vi "Main Page.vi"(8 "error in (no error)":errorcluster, 11 "Node Ptr":T1 format="%.0x") -> (0 "error out":errorcluster)   [LabVIEW 2020, in "FPGA Addon System Explorer.lvlib"]
uses:
  FPGA Addon System Explorer.lvlib
  <vilib>/NI VeriStand/Custom Device API/Custom Device API.lvlib
  Addon Shared/FPGA Addon Shared.lvlib
  Addon Shared/Types/FG Action.ctl
  <vilib>/NI/NI VeriStand Hardware Resource Discovery/NIVS Hardware Discovery.lvlib
  <vilib>/NI/NI VeriStand Hardware Resource Discovery/_Types/Filter Type.ctl
  <vilib>/NI VeriStand/Custom Device API/Custom Device Item Ref.ctl
panel:
  in  "Refresh bitfile":bool
  out "Group?":bool
  in  "RIO Browse":bool
  out "Version":string
  in  "SHDocVw.IWebBrowser":refnum<k7>(container)
  in  "RIO Device":string
  in  "Bitfile path":path
  in  "Header 2":cluster{"Section Name":string}={"Section Name"="FPGA Settings"}
  in  "Header":cluster{"Section Name":string}={"Section Name"="Addon Settings"}
  in  "Description":string
  in  "Name":string
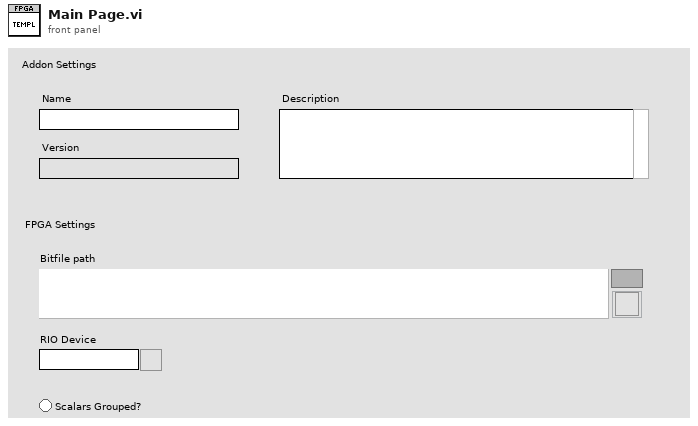
[diagram p1: front panel]
types:
  T1 = typedef "Custom Device API.lvlib/Custom Device Item Ref.ctl" = u64
  T2 = typedef "FPGA Addon Shared.lvlib/FG Action.ctl" = enum8{"GET", "SET"}
  T3 = typedef "FPGA Addon Shared.lvlib/FPGA Settings.ctl" = cluster{"Bitfile path":path, "RIO Device Address":string, "Group":bool}
  T4 = typedef "Custom Device API.lvlib/Custom Device Item Info.ctl" = cluster{"Name":string, "Is Channel":bool, "GUID":string, "Is Waveform":bool}
  T5 = typedef "NIVS Hardware Discovery.lvlib/Filter Type.ctl" = enum16{"Device Category", "Product Name", "Ethernet", "XNET", "VISA", "FPGA", "EtherCAT Master", "DAQmx", "GPIB", "Serial"}
  T6 = typedef "Custom Device API.lvlib/Custom Device Commands.ctl" = enum16{"Default", "Item renamed", "Shutdown", "Dynamic button pressed"}
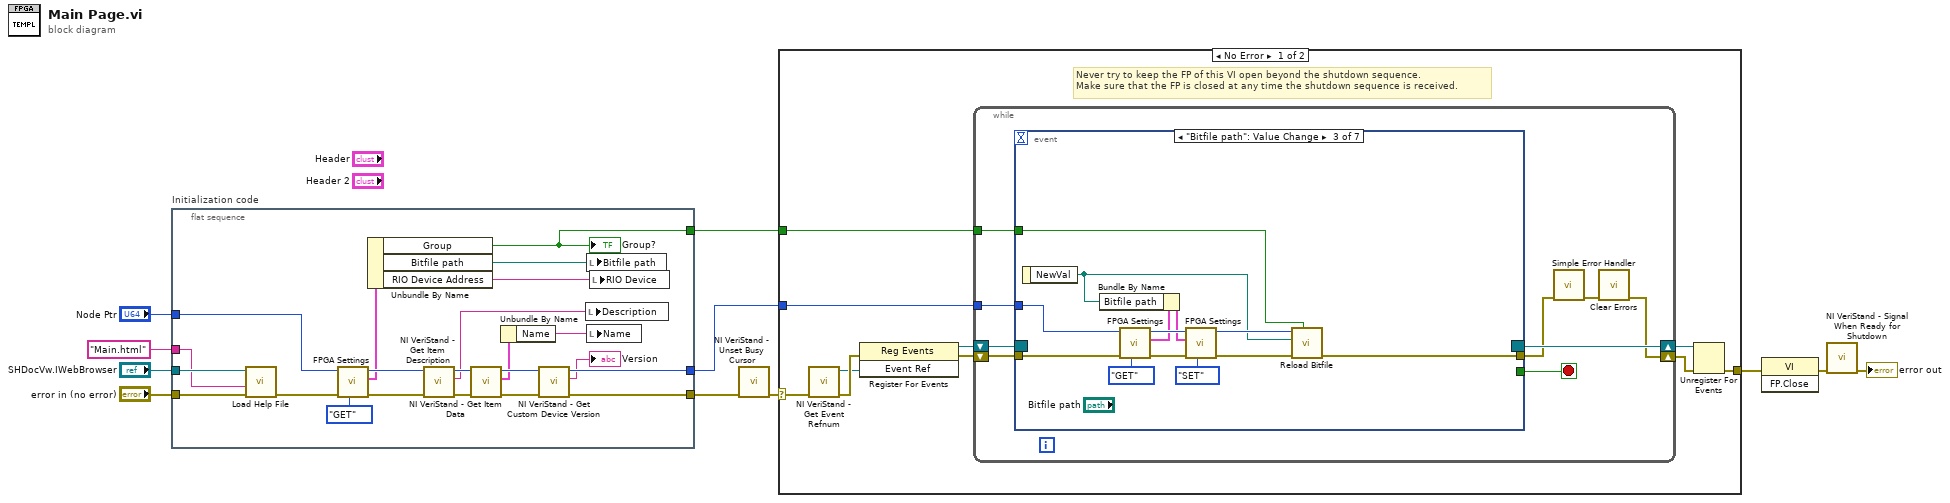
[diagram p0: block diagram]
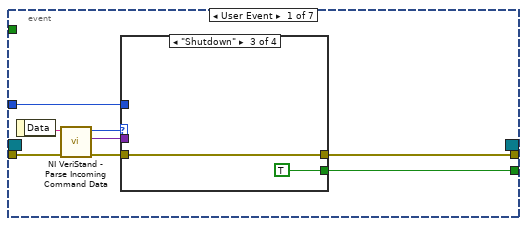
[diagram p2: hidden frame]
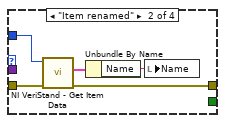
[diagram p4: hidden frame]
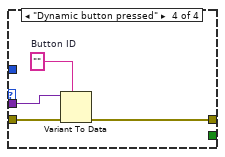
[diagram p5: hidden frame]
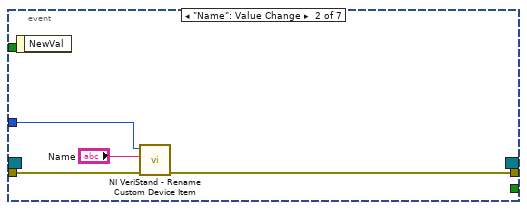
[diagram p6: hidden frame]
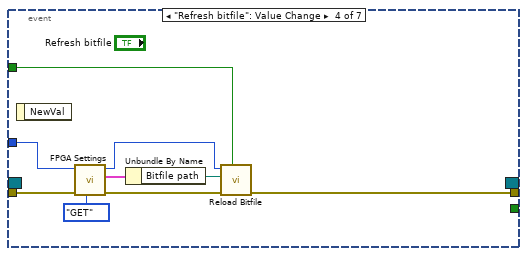
[diagram p7: hidden frame]
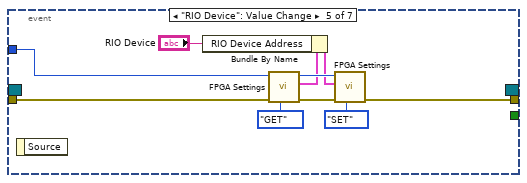
[diagram p8: hidden frame]
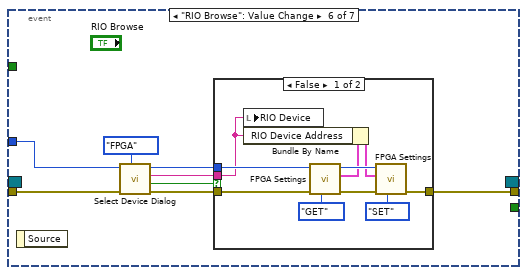
[diagram p9: hidden frame]
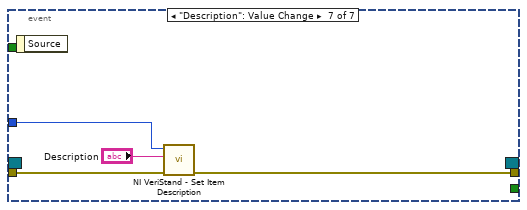
[diagram p11: hidden frame]
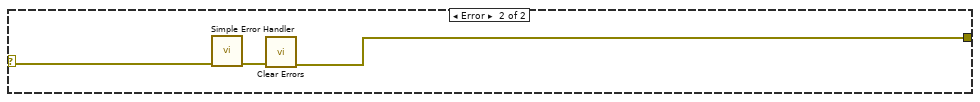
[diagram p12: hidden frame]
diagram:
  n1 = flat-sequence "Initialization code" {
    tunnel: "error in (no error)" -> [w27]
    tunnel: "Node Ptr" -> [w24]
    tunnel: [w15] -> w7
    tunnel: [w16] -> w4
    tunnel: "SHDocVw.IWebBrowser" -> [w26]
    tunnel: "Main.html" ("HTML File") -> [w25]
    tunnel: [w12] -> w1
    frame #0 {
      n2 = call "Load Help File.vi"("error in (no error)"=w27, "HTML File to Load"=w25, "SHDocVw.IWebBrowser2"=w26) -> ("error out"=w23:errorcluster)  [unwired: 8 in]
      n3 = call "FPGA Settings.vi"("Action"=FG_Action."GET", "error in (no error)"=w23, "Item Ref"=w24) -> ("error out"=w21:errorcluster, "FPGA Settings"=w19:T3, "Item Ref out"=w22:T1)  [unwired: 6 in]
      n4 = Unbundle By Name(w19) -> ("Group"=w12:bool, "Bitfile path"=w17:path, "RIO Device Address"=w18:string)
      "Group?" <- w12
      n5 = call <vilib>:"NI VeriStand - Get Item Description.vi"("error in (no error)"=w21, "Item Ref in"=w22) -> ("error out"=w30:errorcluster, "Description"=w31:string, "Item Ref out"=w32:T1)  [unwired: 7 out]
      n6 = call <vilib>:"NI VeriStand - Get Item Data.vi"("error in (no error)"=w30, "Item Ref in"=w32) -> ("error out"=w14:errorcluster, "Item Info"=w29:T4, "Item Ref out"=w33:T1)  [unwired: 7 out]
      n7 = Unbundle By Name(w29) -> ("Name"=w28:string)
      n8 = call <vilib>:"NI VeriStand - Get Custom Device Version.vi"("error in (no error)"=w14, "Device Ref in"=w33) -> ("error out"=w15:errorcluster, "Value"=→"Version":string, "Device Ref out"=w16:T1)  [unwired: 7 in]
      n9 = local write "Description"(w31) -> ()
      n10 = local write "Bitfile path"(w17) -> ()
      n11 = local write "Name"(w28) -> ()
      n12 = local write "RIO Device"(w18) -> ()
    }
  }
  n13 = call <vilib>:"NI VeriStand - Unset Busy Cursor.vi"("error in (no error)"=w7) -> ("error out"=w6:errorcluster)  [unwired: 10 out]
  n14 = case shown="No Error" w6 {
    selector: w6 -> [w35 w134]
    tunnel: [w40 w132] -> w11
    tunnel: w4 -> [w36 _]
    tunnel: w1 -> [w34 _]
    frame No Error {
      # "Never try to keep the FP of this VI open beyond the shutdown sequence.\nMake sure that the FP is closed at any time the shutdown sequence is received."
      n15 = call <vilib>:"NI VeriStand - Get Event Refnum.vi"("error in (no error)"=w35) -> ("error out"=w43:errorcluster, "Event Ref"=w39:refnum<user-event>)  [unwired: 9 out]
      n16 = register-events(error in=w43, w39) -> (reference out=w37:refnum<event-registration>, error out=w38:errorcluster)  [unwired: 1 in]
      n17 = while {
        tunnel: w36 -> [w48]
        shift-right: [w45] -> w41
        shift-left: w38 -> [w51]
        shift-right: [w52] -> w42
        shift-left: w37 -> [w50]
        tunnel: w34 -> [w44]
        stop <- w49 stop-if-true
        n18 = event shown="[2] \"Bitfile path\": Value Change" {
          selector: w50 -> [_ _ _ _ _ _ _]
          dyn-events: [_ _ _ _ _ _ _] -> w52
          timeout: _ -> [_ _ _ _ _ _ _]
          tunnel: w51 -> [w60 w76 w85 w95 w102 w114 w130]
          tunnel: [w56 _ _ _ _ _ _] -> w49
          tunnel: [w55 w75 w79 w93 w99 w116 w129] -> w47
          tunnel: w48 -> [w54 w74 w84 w94 w101 w115 w131]
          tunnel: w44 -> [_ _ w81 w92 _ _ _]
          event User Event {
            n19 = event-data() -> ("Data"=w59:string)  [unwired: 1 out]
            n20 = call <vilib>:"NI VeriStand - Parse Incoming Command Data.vi"("error in (no error)"=w60, "Incoming data"=w59) -> ("error out"=w58:errorcluster, "Outgoing data"=w53:variant, "Action"=w57:T6)  [unwired: 7 out]
            n21 = case shown="\"Shutdown\"" w57 {
              tunnel: w58 -> [w61 w66 w67 w72]
              tunnel: [_ _ TRUE _] -> w56
              tunnel: [w61 w63 w67 w69] -> w55
              tunnel: w54 -> [_ w65 _ _]
              tunnel: w53 -> [_ _ _ w71]
              frame "Default", Default {
              }
              frame "Item renamed" {
                n22 = call <vilib>:"NI VeriStand - Get Item Data.vi"("error in (no error)"=w66, "Item Ref in"=w65) -> ("error out"=w63:errorcluster, "Item Info"=w64:T4)  [unwired: 8 out]
                n23 = Unbundle By Name(w64) -> ("Name"=w62:string)
                n24 = local write "Name"(w62) -> ()
              }
              frame "Shutdown" {
              }
              frame "Dynamic button pressed" {
                w70 = ""  # Button ID
                n25 = Variant To Data(error in=w72, type=w70, Variant=w71) -> (error out=w69:errorcluster)  [unwired: 1 out]
              }
            }
          }
          event "Name": Value Change {
            n26 = event-data() -> ()  [unwired: 2 out]
            n27 = call <vilib>:"NI VeriStand - Rename Custom Device Item.vi"("error in (no error)"=w76, "New Name"="Name", "Item Ref in"=w74) -> ("error out"=w75:errorcluster)  [unwired: 1 in, 7 out]
          }
          event "Bitfile path": Value Change {
            n28 = event-data() -> ("NewVal"=w77:path)  [unwired: 1 out]
            n29 = call "FPGA Settings.vi"("Action"=FG_Action."GET", "error in (no error)"=w85, "Item Ref"=w84) -> ("error out"=w86:errorcluster, "FPGA Settings"=w83:T3, "Item Ref out"=w87:T1)  [unwired: 6 in]
            n30 = Bundle By Name(cluster=w83, "Bitfile path"=w77) -> (w82:T3)
            n31 = call "FPGA Settings.vi"("Action"=FG_Action."SET", "error in (no error)"=w86, "FPGA Settings"=w82, "Item Ref"=w87) -> ("error out"=w80:errorcluster, "Item Ref out"=w78:T1)  [unwired: 5 in, 1 out]
            n32 = call "Reload Bitfile.vi"("Group"=w81, "error in (no error)"=w80, "NewVal"=w77, "Item Ref in"=w78) -> ("error out"=w79:errorcluster)  [unwired: 6 in, 1 out]
          }
          event "Refresh bitfile": Value Change {
            n33 = event-data() -> ()  [unwired: 2 out]
            n34 = call "FPGA Settings.vi"("Action"=FG_Action."GET", "error in (no error)"=w95, "Item Ref"=w94) -> ("error out"=w96:errorcluster, "FPGA Settings"=w91:T3, "Item Ref out"=w97:T1)  [unwired: 6 in]
            n35 = Unbundle By Name(w91) -> ("Bitfile path"=w90:path)
            n36 = call "Reload Bitfile.vi"("Group"=w92, "error in (no error)"=w96, "NewVal"=w90, "Item Ref in"=w97) -> ("error out"=w93:errorcluster)  [unwired: 6 in, 1 out]
          }
          event "RIO Device": Value Change {
            n37 = event-data() -> ()  [unwired: 2 out]
            n38 = call "FPGA Settings.vi"("Action"=FG_Action."GET", "error in (no error)"=w102, "Item Ref"=w101) -> ("error out"=w105:errorcluster, "FPGA Settings"=w104:T3, "Item Ref out"=w106:T1)  [unwired: 6 in]
            n39 = Bundle By Name(cluster=w104, "RIO Device Address"="RIO Device") -> (w103:T3)
            n40 = call "FPGA Settings.vi"("Action"=FG_Action."SET", "error in (no error)"=w105, "FPGA Settings"=w103, "Item Ref"=w106) -> ("error out"=w99:errorcluster)  [unwired: 5 in, 2 out]
          }
          event "RIO Browse": Value Change {
            n41 = event-data() -> ()  [unwired: 2 out]
            n42 = call <vilib>:"Select Device Dialog.vi"("Filter Type"=Filter_Type."FPGA", "error in (no error)"=w114, "Item Ref in"=w115) -> ("error out"=w112:errorcluster, "Cancelled?"=w111:bool, "Selected Alias"=w110:string, "Item Ref out"=w113:T1)  [unwired: 5 in]
            n43 = case shown="False" w111 {
              tunnel: w112 -> [w120 w127]
              tunnel: w113 -> [w119 _]
              tunnel: [w118 w127] -> w116
              tunnel: w110 -> [w117 _]
              frame False {
                n44 = local write "RIO Device"(w117) -> ()
                n45 = call "FPGA Settings.vi"("Action"=FG_Action."GET", "error in (no error)"=w120, "Item Ref"=w119) -> ("error out"=w123:errorcluster, "FPGA Settings"=w122:T3, "Item Ref out"=w124:T1)  [unwired: 6 in]
                n46 = Bundle By Name(cluster=w122, "RIO Device Address"=w117) -> (w121:T3)
                n47 = call "FPGA Settings.vi"("Action"=FG_Action."SET", "error in (no error)"=w123, "FPGA Settings"=w121, "Item Ref"=w124) -> ("error out"=w118:errorcluster)  [unwired: 5 in, 2 out]
              }
              frame True {
              }
            }
          }
          event "Description": Value Change {
            n48 = event-data() -> ()  [unwired: 2 out]
            n49 = call <vilib>:"NI VeriStand - Set Item Description.vi"("error in (no error)"=w130, "Description"="Description", "Item Ref in"=w131) -> ("error out"=w129:errorcluster)  [unwired: 8 out]
          }
        }
        n50 = call <vilib>:"Simple Error Handler.vi"("error in (no error)"=w47) -> ("error out"=w46:errorcluster)  [unwired: 1 in, 7 out]
        n51 = call <vilib>:"Clear Errors.vi"("error in (no error)"=w46) -> ("error out"=w45:errorcluster)  [unwired: 1 in, 5 out]
      }
      n52 = Unregister For Events(event registration refnum=w42, error in=w41) -> (error out=w40:errorcluster)
    }
    frame Error {
      n53 = call <vilib>:"Simple Error Handler.vi"("error in (no error)"=w134) -> ("error out"=w133:errorcluster)  [unwired: 1 in, 7 out]
      n54 = call <vilib>:"Clear Errors.vi"("error in (no error)"=w133) -> ("error out"=w132:errorcluster)  [unwired: 1 in, 5 out]
    }
  }
  n55 = invoke class="VI" method="FP.Close"(error in=w11) -> (error out=w10:errorcluster)  [unwired: 2 in, 2 out]
  n56 = call <vilib>:"NI VeriStand - Signal When Ready for Shutdown.vi"("error in (no error)"=w10) -> ("error out"=→"error out":errorcluster)  [unwired: 10 out]
